vi "Init M5Stack8ChPWM.vi"(8 "error in (no error)":errorcluster, 11 "M5Stack I2C 8Ch Servo in":refnum<class "M5Stack I2C 8Ch Servo.lvclass">) -> (0 "error out":errorcluster, 3 "M5Stack I2C 8Ch Servo out":refnum<class "M5Stack I2C 8Ch Servo.lvclass">)   [LabVIEW 2020, in "CTI-Peripheral.lvlib" / "M5Stack I2C 8Ch Servo.lvclass"]
uses:
  M5Stack I2C 8Ch Servo.lvclass
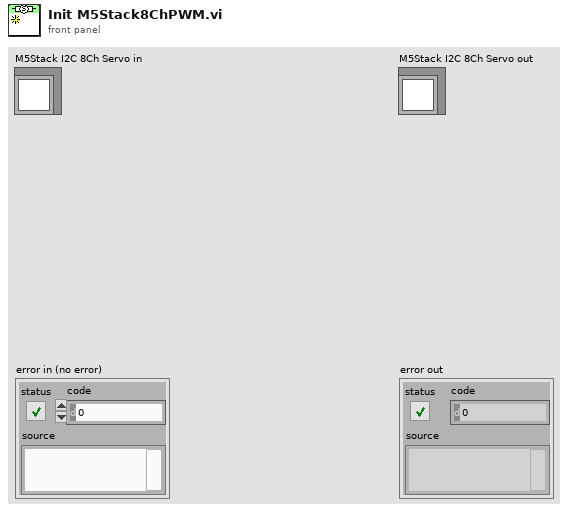
[diagram p1: front panel]
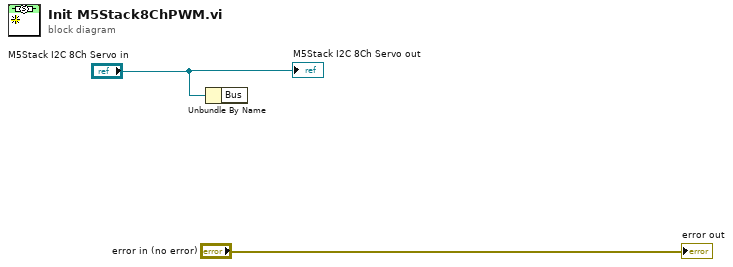
[diagram p0: block diagram]
diagram:
  n1 = Unbundle By Name("M5Stack I2C 8Ch Servo in") -> ()  [unwired: 1 out]
  "error out" <- "error in (no error)"
  "M5Stack I2C 8Ch Servo out" <- "M5Stack I2C 8Ch Servo in"
